vi "G-CLI Help Message--constant.vi"() -> (3 "G-CLI Help Message":string)   [LabVIEW 2026]
doc: "Help message to display through g-cli."
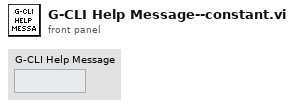
[diagram p1: front panel]
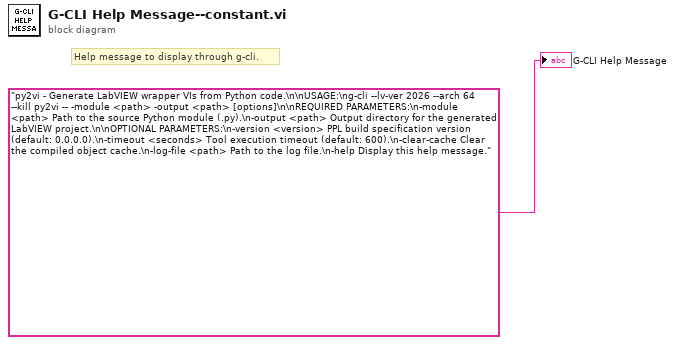
[diagram p0: block diagram]
diagram:
  # "Help message to display through g-cli."
  "G-CLI Help Message" <- "py2vi - Generate LabVIEW wrapper VIs from Python code.\n\nUSAGE:\ng-cli --lv-ver 2026 --arch 64 --kill py2vi -- -module <path> -output <path> [options]\n\nREQUIRED PARAMETERS:\n-module <path> Path to the source Python module (.py).\n-output <path> Output directory for the generated LabVIEW project.\n\nOPTIONAL PARAMETERS:\n-version <version> PPL build specification version (default: 0.0.0.0).\n-timeout <seconds> Tool execution timeout (default: 600).\n-clear-cache Clear the compiled object cache.\n-log-file <path> Path to the log file.\n-help Display this help message."
